vi "Own20261012_CleanDiagram.vi"() -> ()   [LabVIEW 2024]
doc: "本范例使用LabVIEW脚本功能以编程方式创建一个功能型VI，调用程序框图整理，然后运行。\n\n本VI中包含While循环、一个随机函数和一个波形图表。"
panel:
  out "error out":errorcluster caption="错误输出"
  in  "target_path":path
  # "概述：演示如何使用VI脚本通过编程在程序框图上创建一个随机数带状图。\n操作步骤：\n运行VI。以编程方式创建一个新的随机数带状图表VI，整理VI的程序框图并运行VI。"
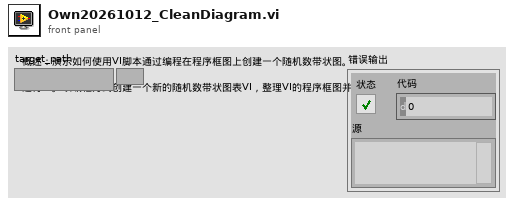
[diagram p1: front panel]
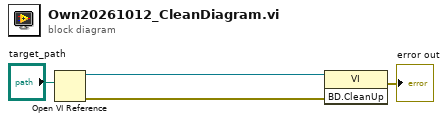
[diagram p0: block diagram]
diagram:
  n1 = Open VI Reference(vi path="target_path") -> (vi reference=w3:refnum<vi>, error out=w2:errorcluster)  [unwired: 5 in]
  n2 = invoke class="VI" method="BD.CleanUp"(reference=w3, error in=w2) -> (error out=→"error out":errorcluster)  [unwired: 1 in, 2 out]
